vi "FuncVI-scancdb.vi"(5 "InstanceRef":T2, 9 "arg list":T1[](array[typedef]) {"num" format="%.2f"}) -> (0 "error out":bool, 3 "result":T1 {"num" format="%.2f"})   [LabVIEW 2021]
doc: "::: CalcExpress Toolkit :::\nCopyright (c) 2000-2026 Konstantin Shifershteyn. All rights reserved."
uses:
  cetypes.llb/CalcExpress Function Argument Info.ctl
  cetypes.llb/CalcExpress Instance RefNum.ctl
panel:
  in  "max arg num":i32=3
  in  "min arg num":i32=1
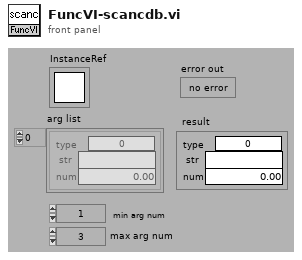
[diagram p1: front panel]
types:
  T1 = typedef "CalcExpress Function Argument Info.ctl" = cluster{"type":u32, "str":string, "num":dbl}
  T2 = typedef "CalcExpress Instance RefNum.ctl" = refnum<k1>
  T3 = cluster{"index":i32, "data type":enum32{"String", "DBL Number", "identifier", "1D Array of DBL", "2D Array of DBL", "CDB Number", "1D Array of CDB", "2D Array of CDB", "1D Array of String", "2D Array of String", "Unknown data type"}, "default num":dbl, "default str":string}[]
  T4 = enum32{"String", "DBL Number", "identifier", "1D Array of DBL", "2D Array of DBL", "CDB Number", "1D Array of CDB", "2D Array of CDB", "1D Array of String", "2D Array of String", "Unknown data type"}
  T5 = cluster{"data type":enum32{"String", "DBL Number", "identifier", "1D Array of DBL", "2D Array of DBL", "CDB Number", "1D Array of CDB", "2D Array of CDB", "1D Array of String", "2D Array of String", "Unknown data type"}, "data string":string, dbl}
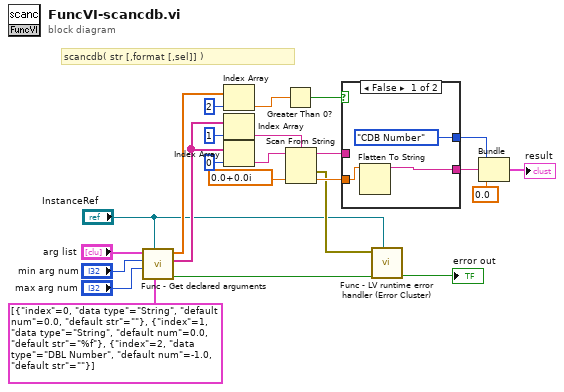
[diagram p0: block diagram]
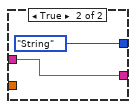
[diagram p2: hidden frame]
diagram:
  # "scancdb( str [,format [,sel]] )"
  n1 = call "Func - Get declared arguments.vi"("arg descriptors"=T3 [{"index"=0, "data type"=enum."String", "default num"=0.0, "default str"=""}, {"index"=1, "data type"=enum."String", "default num"=0.0, "default str"="%f"}, {"index"=2, "data type"=enum."DBL Number", "default num"=-1.0, "default str"=""}] ("args descriptors"), "InstanceRef"="InstanceRef", "max arg num"="max arg num", "min arg num"="min arg num", "arg list"="arg list") -> ("error out"=w2:bool, "str list"=w20:string[], "num list"=w15:dbl[])  [unwired: 3 in, 1 out]
  n2 = Index Array(array=w15, index=2) -> (element=w7:dbl)
  n3 = Index Array(array=w20, index=1) -> (element=w19:string)
  n4 = Index Array(array=w20, index=0) -> (element=w18:string)
  n5 = Greater Than 0?(x=w7) -> (x > 0?=w12:bool)
  n6 = Scan From String(format string=w19, input string=w18, default 1=cdb 0.0+0.0i) -> (remaining string=w11:string, error out=w4:errorcluster, output 1=w10:cdb)  [unwired: 2 in, 1 out]
  n7 = case shown="False" w12 {
    tunnel: w11 -> [_ w29]
    tunnel: w10 -> [w27 _]
    tunnel: [w26 w29] -> w9
    tunnel: [T4."CDB Number" ("data type") T4."String" ("data type")] -> w8
    frame False {
      n8 = Flatten To String(anything=w27) -> (data string=w26:string)  [unwired: 3 in, 2 out]
    }
    frame True {
    }
  }
  n9 = call "Func - LV runtime error handler (Error Cluster).vi"("InstanceRef"="InstanceRef", "error in"=w2, "LabVIEW error"=w4) -> ("error out"=→"error out":bool)  [unwired: 3 in, 3 out]
  n10 = Bundle("data type"=w8, "data string"=w9, 0.0) -> (→"result":T5)  [unwired: 1 in]
